vi "FuncVI2-ScriptPath.vi"(4 "CSE RefNum":T1, 5 "InstanceRef":T3, 9 "arg list":T2[](array[typedef]) {"num" format="%.2f"}) -> (0 "error out":bool, 3 "result":T2 {"num" format="%.2f"})   [LabVIEW 2021]
doc: "::: CalcExpress Toolkit :::\nCopyright (c) 2000-2026 Konstantin Shifershteyn. All rights reserved."
uses:
  cetypes.llb/CalcExpress Function Argument Info.ctl
  cetypes.llb/CalcExpress Instance RefNum.ctl
  cse.llb/CSE Instance RefNum.ctl
panel:
  in  "max arg num":i32=1
  in  "min arg num":i32
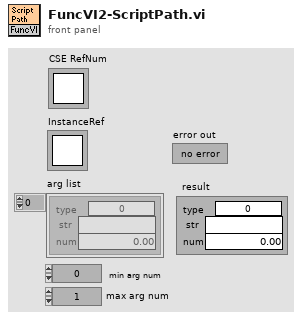
[diagram p1: front panel]
types:
  T1 = typedef "CSE Instance RefNum.ctl" = refnum<k1>
  T2 = typedef "CalcExpress Function Argument Info.ctl" = cluster{"type":u32, "str":string, "num":dbl}
  T3 = typedef "CalcExpress Instance RefNum.ctl" = refnum<k1>
  T4 = cluster{"index":i32, "data type":enum32{"String", "DBL Number", "identifier", "1D Array of DBL", "2D Array of DBL", "CDB Number", "1D Array of CDB", "2D Array of CDB", "1D Array of String", "2D Array of String", "Unknown data type"}, "default num":dbl, "default str":string}[]
  T5 = enum32{"String", "DBL Number", "identifier", "1D Array of DBL", "2D Array of DBL", "CDB Number", "1D Array of CDB", "2D Array of CDB", "1D Array of String", "2D Array of String", "Unknown data type"}
  T6 = cluster{"level":i32, "Caller CSE RefNum":T1, "Callee CSE RefNum":T1}
  T7 = cluster{"type: use this constant to specify a predefined type code":enum32{"String", "DBL Number", "identifier", "1D Array of DBL", "2D Array of DBL", "CDB Number", "1D Array of CDB", "2D Array of CDB", "1D Array of String", "2D Array of String", "Unknown data type"}, string, dbl}
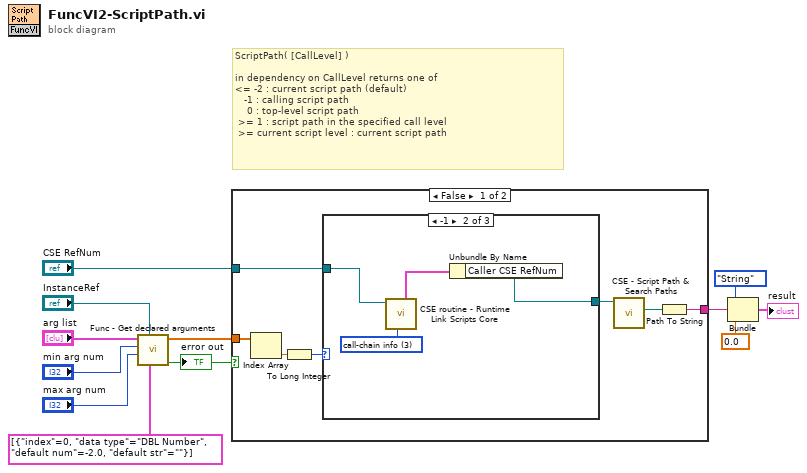
[diagram p0: block diagram]
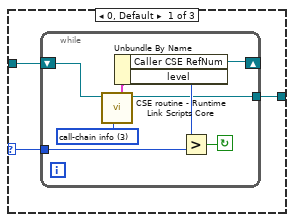
[diagram p2: hidden frame]
diagram:
  # "ScriptPath( [CallLevel] ) \n\nin dependency on CallLevel returns one of\n<= -2 : current script path (default)\n   -1 : calling script path\n    0 : top-level script path\n >= 1 : script path in the specified call level\n >= current script level : current script path"
  n1 = call "Func - Get declared arguments.vi"("arg descriptors"=T4 [{"index"=0, "data type"=enum."DBL Number", "default num"=-2.0, "default str"=""}], "InstanceRef"="InstanceRef", "max arg num"="max arg num", "min arg num"="min arg num", "arg list"="arg list") -> ("error out"=w5:bool, "num list"=w3:dbl[])  [unwired: 3 in, 2 out]
  "error out" <- w5
  n2 = case shown="False" w5 {
    tunnel: w3 -> [w19 _]
    tunnel: [w14 _] -> w2
    tunnel: "CSE RefNum" -> [w13 _]
    frame False {
      n3 = Index Array(array=w19) -> (element=w18:dbl)  [unwired: 1 in]
      n4 = To Long Integer(number=w18) -> (32bit integer=w17:i32)
      n5 = case shown="-1" w17 {
        selector: w17 -> [w21 _ _]
        tunnel: w13 -> [w22 w32 w35]
        tunnel: [w20 w31 w35] -> w15
        frame 0, Default {
          n6 = while {
            shift-right: [w27] -> _
            shift-left: w22 -> [w28]
            tunnel: w21 -> [w26]
            tunnel: [w23] -> w20
            stop <- w24 continue-if-true
            w30 = 3 items=["save vi path", "link to caller", "delink of caller", "call-chain info"] ("action")
            n7 = call "CSE routine - Runtime Link Scripts Core.vi"("action"=w30, "CSE RefNum"=w28) -> ("dup CSE RefNum"=w23:T1, "call-chain info"=w29:T6)  [unwired: 4 in, 4 out]
            n8 = Unbundle By Name(w29) -> ("Caller CSE RefNum"=w27:T1, "level"=w25:i32)
            n9 = Greater?(x=w25, y=w26) -> (0:w24:bool)
          }
        }
        frame -1 {
          w34 = 3 items=["save vi path", "link to caller", "delink of caller", "call-chain info"] ("action")
          n10 = call "CSE routine - Runtime Link Scripts Core.vi"("action"=w34, "CSE RefNum"=w32) -> ("call-chain info"=w33:T6)  [unwired: 4 in, 5 out]
          n11 = Unbundle By Name(w33) -> ("Caller CSE RefNum"=w31:T1)
        }
        frame ..-2 {
        }
      }
      n12 = call "CSE - Script Path & Search Paths.vi"("CSE RefNum"=w15) -> ("script file path out"=w16:path)  [unwired: 7 in, 3 out]
      n13 = Path To String(path=w16) -> (string=w14:string)
    }
    frame True {
    }
  }
  n14 = Bundle("type: use this constant to specify a predefined type code"=T5."String", w2, 0.0) -> (→"result":T7)  [unwired: 1 in]
